vi "Get Buffer Configuration.vi"(10 "Encoder Data Description":string, 11 "Buffer Configuration in":T1) -> (2 "Type":T4, 3 "Buffer Configuration out":T1)   [LabVIEW 2021, in "CIF_CIPC_Chn.lvclass"]
uses:
  CIF_CIPC_Chn.lvclass
  <vilib>/Utility/Data Type/Type Definitions/Data Type.ctl
  Typedef/Buffer Configuration Data.ctl
  <vilib>/CIF Foundation/CIF CIPC/TypeDefs/Backpressure References.ctl
  <vilib>/CIF Foundation/CIF CIPC/TypeDefs/Backpressure Names.ctl
  <vilib>/CIF Foundation/CIF CIPC/SubVIs/Decode Array Element Data.vi
  <vilib>/Utility/error.llb/Trim Whitespace.vi
  CIF_CIPC_Chn.lvclass/CIF_CIPC_Chn.ctl
  <vilib>/CIF Foundation/CIF CIPC/CIF_NI_CIPC.lvlib
  <vilib>/Utility/Data Type/NI_Data Type.lvlib
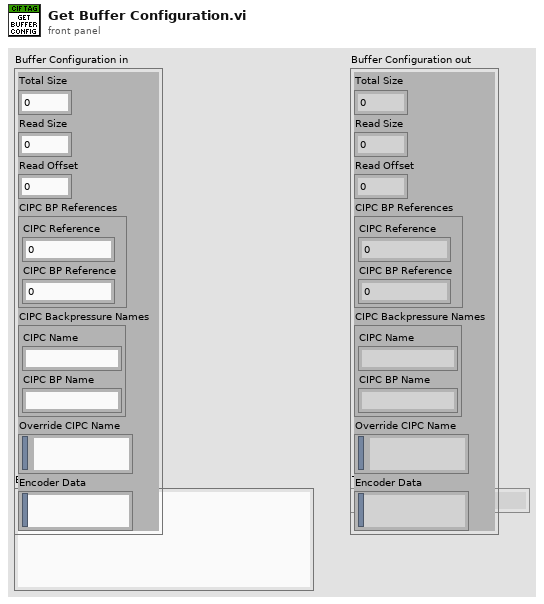
[diagram p1: front panel]
types:
  T1 = typedef "CIF_CIPC_Chn.lvclass/Buffer Configuration Data.ctl" = cluster{"Total Size":u32, "Read Size":u32, "Read Offset":u32, "CIPC BP References":T2, "CIPC Backpressure Names":T3, "Override CIPC Name":string, "Encoder Data":string}
  T2 = typedef "CIF_NI_CIPC.lvlib/Backpressure References.ctl" = cluster{"CIPC Reference":u64, "CIPC BP Reference":u64}
  T3 = typedef "CIF_NI_CIPC.lvlib/Backpressure Names.ctl" = cluster{"CIPC Name":string, "CIPC BP Name":string}
  T4 = typedef "NI_Data Type.lvlib/Data Type.ctl" = enum8{"Invalid Type", "Void", "I8", "I16", "I32", "I64", "U8", "U16", "U32", "U64", "Single Float", "Double Float", "Extended Float", "Single Complex", "Double Complex", "Extended Complex", "Enum U8", "Enum U16", "Enum U32", "Enum U64", "Single Float With Unit", "Double Float With Unit", "Extended Float With Unit", "Single Complex with Unit", "Double Complex with Unit", "Extended Complex with Unit", "Boolean", "String", "Path", "Picture", "Tag", "Array", "Cluster", "Variant", "LV Variant", "Waveform", "Timestamp", "Digital Waveform", "Digital Data", "ExpressData", "Refnum", "External Data", "VI", "Poly VI", "LabVIEW Class Instance", "Fixed Point", "Set Collection", "Map Collection"}
  T5 = typedef "CIF_NI_CIPC.lvlib/Data Encoding.ctl" = cluster{"Data Struct Info":cluster{"Alignment":T6, "Endian":T7, "Array Info":T8, "Total Length (bytes)":i32}, "Data Elements":T9[]}
  T6 = typedef "CIF_NI_CIPC.lvlib/Alignment.ctl" = enum16{"Natural", "Packed"}
  T7 = typedef "DataTypes_CIF_U.lvlib/Endian.ctl" = enum16{"Little Endian", "Big Endian"}
  T8 = typedef "CIF_NI_CIPC.lvlib/Data Struct Array Info.ctl" = cluster{"Array":bool, "Array_Size":i32, "Elem_Size":i32, "Prepended Length":bool}
  T9 = typedef "CIF_NI_CIPC.lvlib/Data Element.ctl" = cluster{"Name":string, "Type":T4, "Size":u32, "Offset":u32}
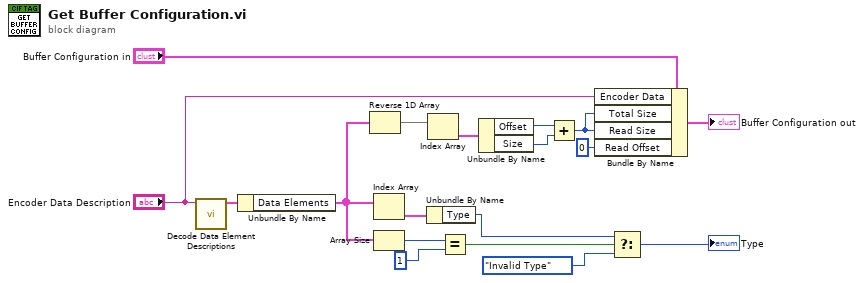
[diagram p0: block diagram]
diagram:
  n1 = call <vilib>:"Decode Data Element Descriptions.vi"("Encoder Data Description"="Encoder Data Description") -> ("Data Encoding"=w2:T5)  [unwired: 10 in]
  n2 = Unbundle By Name(w2) -> ("Data Elements"=w1:T9[])
  n3 = Reverse 1D Array(array=w1) -> (reversed array=w15:T9[])
  n4 = Index Array(array=w1) -> (element=w16:T9)  [unwired: 1 in]
  n5 = Array Size(array=w1) -> (size(s)=w18:i32)
  n6 = Unbundle By Name(w16) -> ("Type"=w7:T4)
  n7 = Index Array(array=w15) -> (element=w14:T9)  [unwired: 1 in]
  n8 = Equal?(x=w18, y=1) -> (x = y?=w6:bool)
  n9 = Unbundle By Name(w14) -> ("Offset"=w13:u32, "Size"=w12:u32)
  n10 = Add(x=w13, y=w12) -> (x+y=w10:u32)
  n11 = Bundle By Name(cluster="Buffer Configuration in", "Encoder Data"="Encoder Data Description", "Total Size"=w10, "Read Size"=w10, "Read Offset"=u32 0) -> (→"Buffer Configuration out":T1)
  n12 = Select(t=w7, s=w6, f=Data_Type."Invalid Type") -> (s? t:f=→"Type":T4)
